vi "move.vi"(8 "error in (no error)":errorcluster, 10 "タは":bool, 11 "移動距離":dbl=155.0 format="%#_13g") -> (0 "error out":errorcluster)   [LabVIEW 2019]
uses:
  <vilib>/Platform/TimedLoop/XDataNode/timing_clust.ctl
  <vilib>/Platform/TimedLoop/XDataNode/nitl_modes.ctl
  <vilib>/Platform/TimedLoop/XDataNode/wakeup.ctl
  <vilib>/platform/TimedLoop/XDataNode/XDataNode.xnode
  <vilib>/Platform/TimedLoop/XDataNode/XDNodeRunTimeDep.lvlib
panel:
  out "誤差":dbl[](array[numeric])=[10401.0, -10400.0]
  in  "Stop Button":bool
  out "x .and. y?":bool=TRUE
  in  "value":dbl=68.0 format="%#_13g"
  out "ENC":dbl[](array[numeric])=[10540.0, -10540.0]
  out "output":dbl[](array[numeric])
  in  "Acc":dbl=0.0015 format="%#_13g"
  in  "Max S":dbl=4.0 format="%#_13g"
  out "Speed":dbl[](graph)
  out "Position":dbl[](graph)
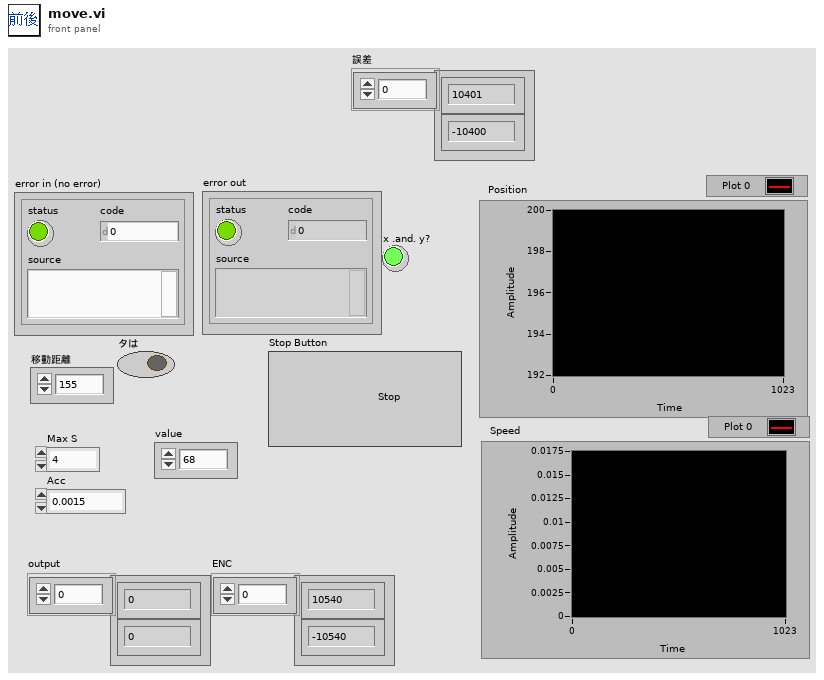
[diagram p1: front panel]
types:
  T1 = typedef "XDNodeRunTimeDep.lvlib/timing_clust.ctl" = cluster{"Expected End [f-1]":u64, "Actual End [f-1]":u64, "Finished Late? [f-1]":bool, "Expected End [i-1]":u64, "Actual End [i-1]":u64, "Finished Late? [i-1]":bool, "Expected Start [i]":u64, "Actual Start [i]":u64, "Expected Start [f]":u64, "Actual Start [f]":u64, "Source Name":string, "Structure Name":string, "Period":i64, "Deadline":i64, "Offset":i64, "Start":i64, "Priority":i32, "Timeout":i32, "Mode":T2, "Wakeup Reason":T3, "Error":errorcluster, "Source Type":string, "Secondary Source Type":string, "Global End Time":u64, "Global Start Time":u64, "Frame Duration":u64, "Iteration Duration":u64, "Assigned CPU":i32, "I/O Scan Engine Mode":u32}
  T2 = typedef "XDNodeRunTimeDep.lvlib/nitl_modes.ctl" = enum32{"No Change", "Process missed periods, maintain original phase", "Discard missed periods, maintain original phase", "Process missed periods, ignore original phase", "Discard missed periods, ignore original phase"}
  T3 = typedef "XDNodeRunTimeDep.lvlib/wakeup.ctl" = enum32{"Normal", "Aborted", "Asynchronous wakeup", "Timing source error", "Timed loop error", "Timeout"}
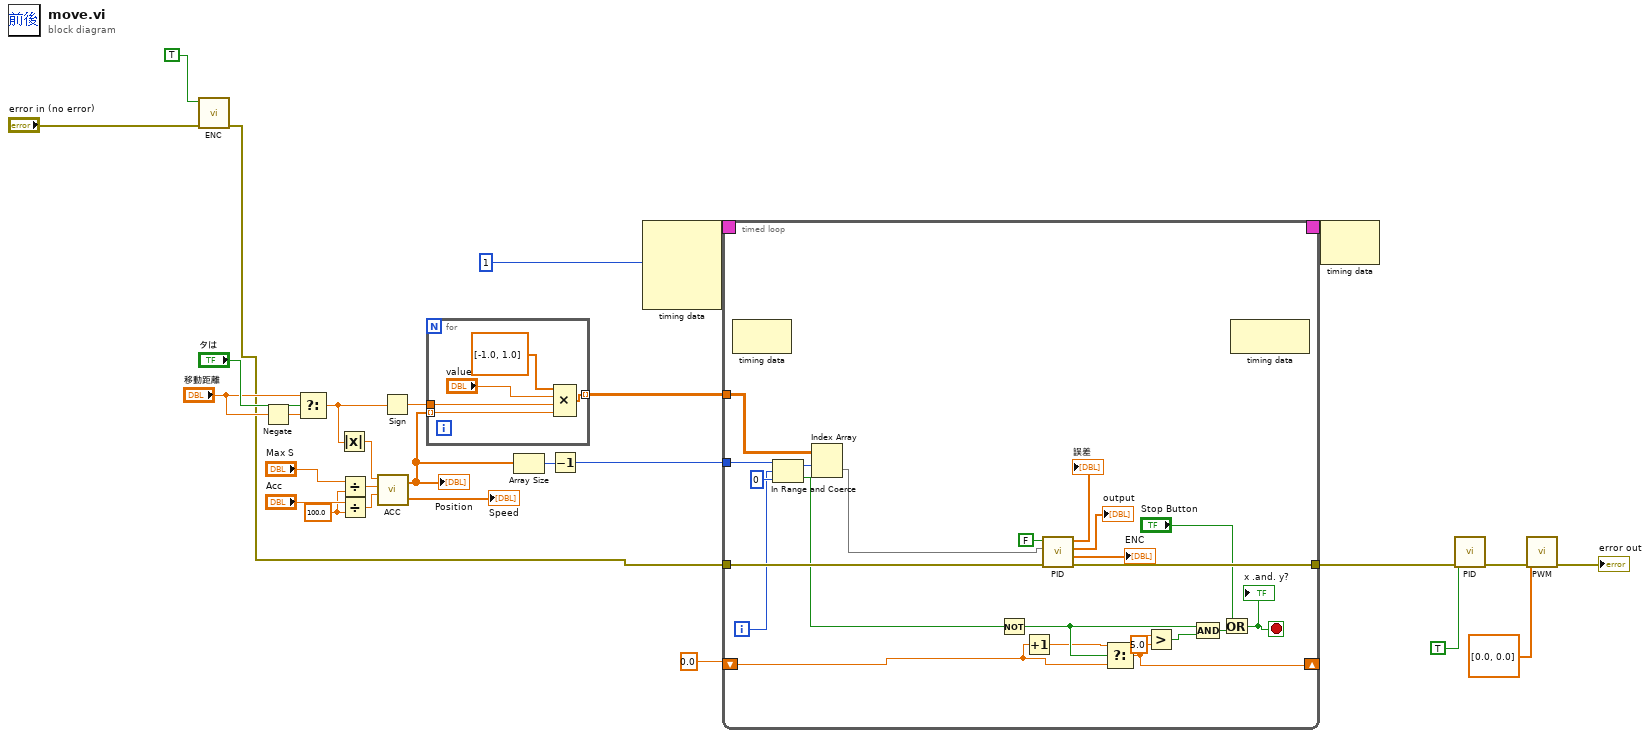
[diagram p0: block diagram]
diagram:
  w11 = 100.0 ("y")
  n1 = call "ENC.vi"("error in (no error)"="error in (no error)", "Reset"=TRUE) -> ("error out"=w1:errorcluster)  [unwired: 6 in, 3 out]
  n2 = Negate(x="移動距離") -> (-x=w5:dbl)
  n3 = Select(t="移動距離", s="タは", f=w5) -> (s? t:f=w7:dbl)
  n4 = Absolute Value(x=w7) -> (abs(x)=w8:dbl)
  n5 = Divide(x="Max S", y=w11) -> (x/y=w14:dbl)
  n6 = Divide(x="Acc", y=w11) -> (x/y=w12:dbl)
  n7 = call "ACC.vi"("Acc"=w12, "Max S"=w14, "Target"=w8) -> ("Speed"=→"Speed":dbl[], "Position"=w23:dbl[])  [unwired: 1 in]
  "Position" <- w23
  n8 = Sign(1:w7) -> (0:w17:dbl)
  n9 = for {
    tunnel: w23 -> [w31] mode=indexing
    tunnel: [w30] -> w21 mode=indexing
    tunnel: w17 -> [w29]
    n10 = Compound Arithmetic op=MULTIPLY(dbl[] [-1.0, 1.0], "value", w29, w31) -> (w30:dbl[])
  }
  n11 = Array Size(array=w23) -> (size(s)=w24:i32)
  n12 = Decrement(x=w24) -> (x-1=w22:i32)
  n13 = node-c288(i64 1 ("Period")) -> (w28:T1)  [unwired: 3 in]
  n14 = timed-loop {
    timing: w28 -> [_]
    timing-out: [_] -> w27
    tunnel: w1 -> [w55]
    tunnel: w22 -> [w53]
    tunnel: w21 -> [w51]
    tunnel: [w48] -> w19
    shift-right: [w38] -> _
    shift-left: 0.0 -> [w39]
    i -> [w46]
    stop <- w44 stop-if-true
    n15 = node-c288() -> ()  [unwired: 1 in, 1 out]
    n16 = In Range and Coerce(upper limit=w53, x=w46, lower limit=0) -> (coerced(x)=w50:i32, In Range?=w49:bool)
    n17 = Index Array(array=w51, index (row)=w50) -> (element=w35:dbl[])  [unwired: 1 in]
    n18 = Not(x=w49) -> (.not. x?=w41:bool)
    n19 = Increment(x=w39) -> (x+1=w40:dbl)
    n20 = call "PID.vi"("error in (no error)"=w55, "目標"=w35, "Reset"=FALSE) -> ("error out"=w48:errorcluster, "ENC"=→"ENC":dbl[], "output"=→"output":dbl[], "誤差"=→"誤差":dbl[])  [unwired: 4 in, 1 out]
    n21 = Select(t=w40, s=w41, f=w39) -> (s? t:f=w38:dbl)
    n22 = Greater?(x=w38, y=5.0) -> (0:w36:bool)
    n23 = Compound Arithmetic op=AND(w41, w36) -> (w43:bool)
    n24 = Or(x="Stop Button", y=w43) -> (x .or. y?=w44:bool)
    "x .and. y?" <- w44
    n25 = node-c288() -> ()  [unwired: 1 in, 1 out]
  }
  n26 = node-c288(w27) -> ()  [unwired: 1 out]
  n27 = call "PID.vi"("error in (no error)"=w19, "Reset"=TRUE ("Reset Counter")) -> ("error out"=w9:errorcluster)  [unwired: 5 in, 4 out]
  n28 = call "PWM.vi"("error in (no error)"=w9, "power"=dbl[] [0.0, 0.0]) -> ("error out"=→"error out":errorcluster)  [unwired: 9 in]
